vi "Get Line Name.vi"(8 "error in":errorcluster, 11 "MB Channel":refnum<class "Modbus Module Channel.lvclass">) -> (0 "error out":errorcluster, 2 "Name":string, 3 "MB Channel":refnum<class "Modbus Module Channel.lvclass">)   [LabVIEW 2015, in "Modbus Module configuration.lvclass"]
uses:
  Modbus Module configuration.lvclass
  module channel/Modbus Module Channel.lvclass
  <vilib>/NI/Tag Bus/tag/tag descriptor.lvclass/tag descriptor.ctl
  <vilib>/NI/Tag Bus/tag/tag descriptor.lvclass
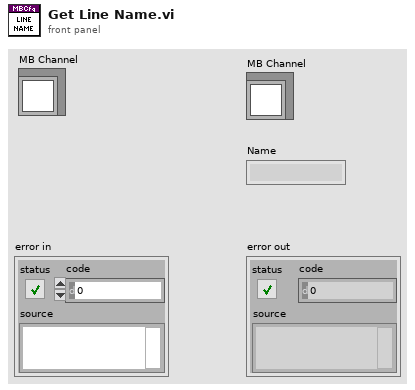
[diagram p1: front panel]
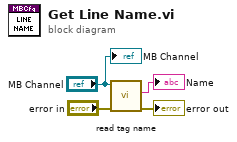
[diagram p0: block diagram]
diagram:
  n1 = call <vilib>:"read tag name.vi"("error in"="error in", "system tag in"="MB Channel") -> ("error out"=→"error out":errorcluster, "name"=→"Name":string)  [unwired: 7 in, 1 out]
  "MB Channel" <- "MB Channel"
